vi "OnCFXMessageReceived_Listener.vi"(4 "Cfx_message":refnum<vi>, 5 "事件数据":T1, 6 "控件引用":refnum<k24>, 7 "事件通用数据":cluster{"事件源":i32, "事件类型":u32, "时间标识":u32}) -> ()   [LabVIEW 2025]
uses:
  CFX_dll/CFX.dll
  SubVI/UT.lib/1.2 log/_log for app error cmd.ctl
panel:
  out "error out":errorcluster caption="错误输出"
  in  "error in":errorcluster caption="错误输入"
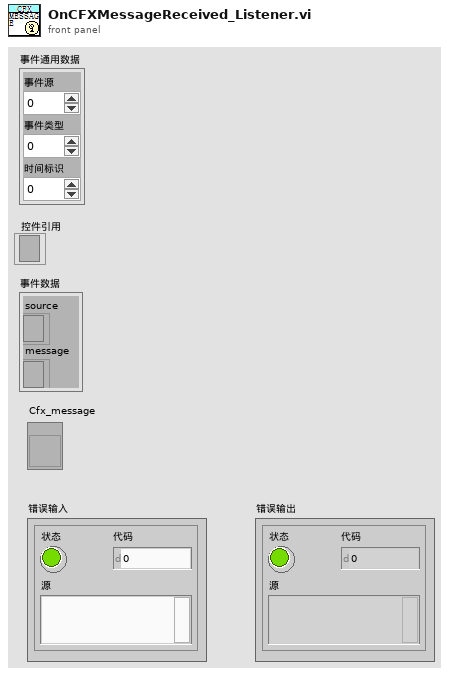
[diagram p1: front panel]
types:
  T1 = cluster{"source":refnum<k24>, "message":refnum<k24>}
  T2 = cluster{"Message_Name":string, "Message_Content":string}
  T3 = typedef "_log for app error cmd.ctl" = enum16{"set str", "show", "init", "save"}
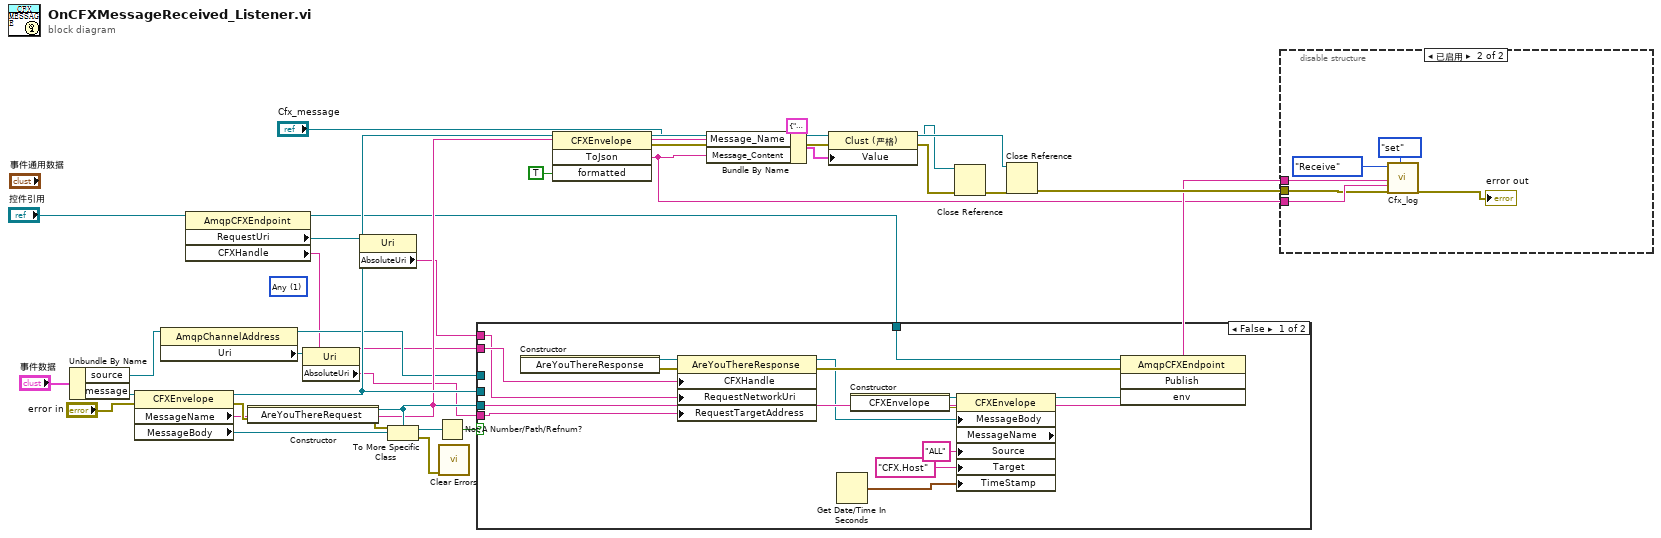
[diagram p0: block diagram]
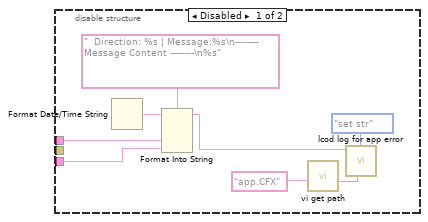
[diagram p2: hidden frame]
diagram:
  (unwired) 1 items=["All", "Any", "Ignore"] ("SupportedTopicQueryType")
  n1 = Unbundle By Name("事件数据") -> ("source"=w29:refnum<k24>, "message"=w31:refnum<k24>)
  n2 = property on="属性节点" class="CFXEnvelope"(reference=w31, error in="error in") -> (reference out=w21:refnum<k24>, error out=w18:errorcluster, "MessageName"=w15:string, "MessageBody"=w28:refnum<k24>)
  n3 = property on="属性节点" class="AmqpChannelAddress"(reference=w29) -> (reference out=w7:refnum<k24>, "Uri"=w3:refnum<k24>)  [unwired: 1 in, 1 out]
  n4 = property on="属性节点" class="AmqpCFXEndpoint"(reference="控件引用") -> (reference out=w1:refnum<k24>, "RequestUri"=w6:refnum<k24>, "CFXHandle"=w5:string)  [unwired: 1 in, 1 out]
  n5 = constructor class="AreYouThereRequest"(error in=w18) -> (reference out=w30:refnum<k24>, error out=w19:errorcluster)  [unwired: 2 in, 1 out]
  n6 = property class="Uri"(reference=w3) -> ("AbsoluteUri"=w2:string)  [unwired: 1 in, 2 out]
  n7 = property class="Uri"(reference=w6) -> ("AbsoluteUri"=w4:string)  [unwired: 1 in, 2 out]
  n8 = To More Specific Class(target class=w30, reference=w28, error in=w19) -> (specific class reference=w27:refnum<k24>, error out=w25:errorcluster)
  n9 = Not A Number/Path/Refnum?(number/path/refnum=w27) -> (NaN/Path/Refnum?=w26:bool)
  n10 = call <vilib>:"Clear Errors.vi"("error in (no error)"=w25) -> ()  [unwired: 5 in, 2 out]
  n11 = case shown="False" w26 {
    tunnel: w21 -> [_ _]
    tunnel: w7 -> [_ _]
    tunnel: w30 -> [_ _]
    tunnel: w5 -> [w44 _]
    tunnel: w4 -> [w43 _]
    tunnel: w2 -> [w42 _]
    tunnel: w1 -> [w41 _]
    frame False {
      n12 = constructor class="AreYouThereResponse"() -> (reference out=w46:refnum<k24>, error out=w45:errorcluster)  [unwired: 3 in, 1 out]
      n13 = property class="AreYouThereResponse"(reference=w46, error in=w45, "CFXHandle"=w44, "RequestNetworkUri"=w43, "RequestTargetAddress"=w42) -> (reference out=w37:refnum<k24>, error out=w40:errorcluster)
      n14 = Get Date/Time In Seconds() -> (seconds since 1Jan1904=w35:timestamp)
      n15 = constructor class="CFXEnvelope"() -> (reference out=w38:refnum<k24>, error out=w39:errorcluster)  [unwired: 3 in, 1 out]
      n16 = property class="CFXEnvelope" props=["MessageBody", "MessageName", "Source", "Target", "TimeStamp"](reference=w38, error in=w39, "MessageBody"=w37, "Source"="ALL", "Target"="CFX.Host", "TimeStamp"=w35) -> (reference out=w36:refnum<k24>)  [unwired: 2 out]
      n17 = invoke class="AmqpCFXEndpoint" method="Publish"(reference=w41, error in=w40, "env"=w36) -> ()  [unwired: 1 in, 4 out]
    }
    frame True {
    }
  }
  n18 = invoke on="调用节点" class="CFXEnvelope" method="ToJson"(reference=w21, "formatted"=TRUE) -> (reference out=w23:refnum<k24>, error out=w24:errorcluster, "ToJson"=w14:string)  [unwired: 2 in, 1 out]
  n19 = Bundle By Name(cluster=T2 {"Message_Name"="", "Message_Content"=""} ("值"), "Message_Name"=w15, "Message_Content"=w14) -> (w9:T2)
  n20 = property class="Clust (严格)"(reference="Cfx_message", error in=w24, "Value"=w9) -> (reference out=w11:refnum<vi>, error out=w13:errorcluster)
  n21 = Close Reference(reference=w11, error in (no error)=w13) -> (error out=w22:errorcluster)
  n22 = Close Reference(reference=w23, error in (no error)=w22) -> (error out=w17:errorcluster)
  n23 = disable-structure shown="已启用" {
    disable-tunnel: w14 -> [w49 w58]
    disable-tunnel: w15 -> [w47 w59]
    disable-tunnel: w17 -> [_ w57]
    frame Disabled {
      n24 = Format Date/Time String() -> (date/time string=w50:string)  [unwired: 3 in]
      n25 = Format Into String(format string="  Direction: %s | Message:%s\n-------- Message Content --------\n%s", initial string=w50, w47, w49) -> (resulting string=w48:string)  [unwired: 2 in, 1 out]
      n26 = call "vi get path.vi"("log name"="app.CFX" ("名称或相对路径")) -> ("log path"=w52:path)  [unwired: 6 in, 4 out]
      n27 = call "lcod log for app error.vi"("appErrFilePath"=w52, "cmd"=_log_for_app_error_cmd."set str", "str in"=w48) -> ()  [unwired: 7 in, 2 out]
    }
    frame Enabled {
      n28 = call "Cfx_log.vi"("R/W"=enum16{"Send", "Receive"}."Receive" ("cmd"), "Message_Name"=w59, "Message_Content"=w58, "error in"=w57, "cmd"=enum16{"init", "set", "save"}."set") -> ("error out"=→"error out":errorcluster)  [unwired: 13 in, 1 out]
    }
  }
